vi "Get stack field.vi"(7 "Is Module?":bool, 8 "error in (no error)":errorcluster, 10 "Field":string, 11 "Stack in":refnum<class "Stack.lvclass">) -> (0 "error out":errorcluster, 1 "Value out":string, 3 "Stack out":refnum<class "Stack.lvclass">)   [LabVIEW 2021, in "Stack.lvclass"]
uses:
  Stack.lvclass
  Stack.lvclass/Stack.ctl
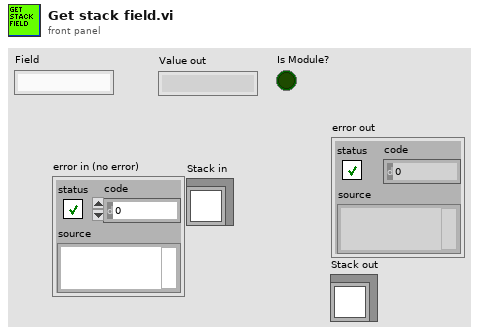
[diagram p1: front panel]
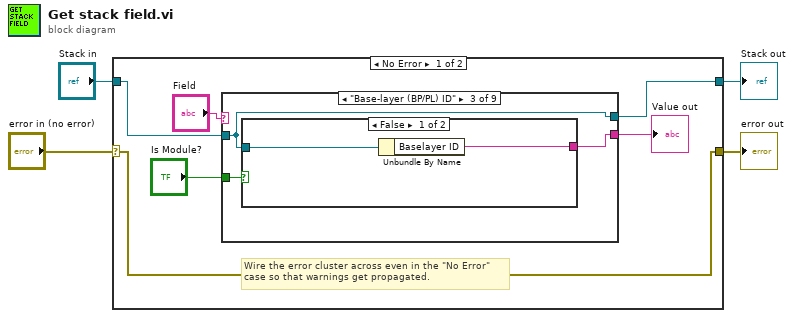
[diagram p0: block diagram]
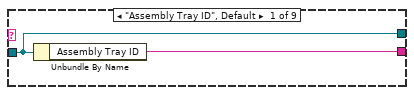
[diagram p2: hidden frame]
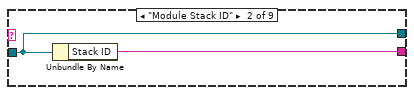
[diagram p3: hidden frame]
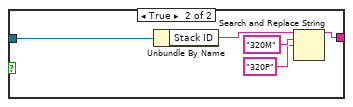
[diagram p4: hidden frame]
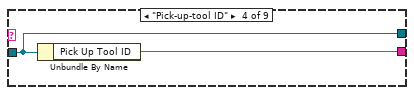
[diagram p5: hidden frame]
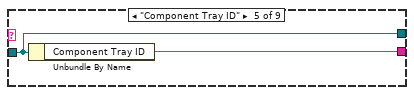
[diagram p6: hidden frame]
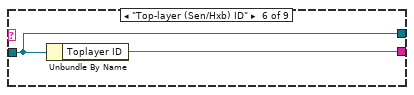
[diagram p7: hidden frame]
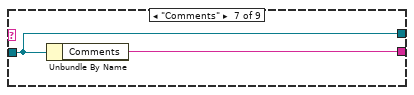
[diagram p8: hidden frame]
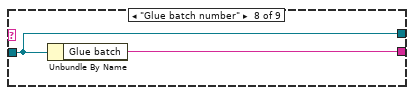
[diagram p9: hidden frame]
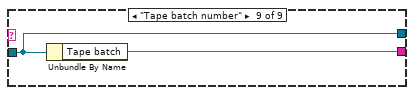
[diagram p10: hidden frame]
diagram:
  n1 = case shown="No Error" "error in (no error)" {
    selector: "error in (no error)" -> [w10 w38]
    tunnel: [w10 w38] -> w3
    tunnel: [w8 w37] -> w1
    tunnel: "Stack in" -> [w9 w37]
    frame No Error {
      # "Wire the error cluster across even in the \"No Error\"\ncase so that warnings get propagated."
      n2 = case shown="\"Base-layer (BP/PL) ID\"" "Field" {
        tunnel: w9 -> [w12 w13 w16 w26 w28 w30 w32 w34 w36]
        tunnel: [w12 w13 w16 w26 w28 w30 w32 w34 w36] -> w8
        tunnel: [w11 w14 w15 w25 w27 w29 w31 w33 w35] -> w6
        tunnel: "Is Module?" -> [_ _ w17 _ _ _ _ _ _]
        frame "Assembly Tray ID", Default {
          n3 = Unbundle By Name(w12) -> ("Assembly Tray ID"=w11:string)
        }
        frame "Module Stack ID" {
          n4 = Unbundle By Name(w13) -> ("Stack ID"=w14:string)
        }
        frame "Base-layer (BP/PL) ID" {
          n5 = case shown="False" w17 {
            tunnel: w16 -> [w19 w24]
            tunnel: [w18 w20] -> w15
            frame False {
              n6 = Unbundle By Name(w19) -> ("Baselayer ID"=w18:string)
            }
            frame True {
              n7 = Unbundle By Name(w24) -> ("Stack ID"=w21:string)
              n8 = Search and Replace String(input string=w21, search string="320M", replace string="320P" ("replace string (\"\")")) -> (result string=w20:string)  [unwired: 5 in, 3 out]
            }
          }
        }
        frame "Pick-up-tool ID" {
          n9 = Unbundle By Name(w26) -> ("Pick Up Tool ID"=w25:string)
        }
        frame "Component Tray ID" {
          n10 = Unbundle By Name(w28) -> ("Component Tray ID"=w27:string)
        }
        frame "Top-layer (Sen/Hxb) ID" {
          n11 = Unbundle By Name(w30) -> ("Toplayer ID"=w29:string)
        }
        frame "Comments" {
          n12 = Unbundle By Name(w32) -> ("Comments"=w31:string)
        }
        frame "Glue batch number" {
          n13 = Unbundle By Name(w34) -> ("Glue batch"=w33:string)
        }
        frame "Tape batch number" {
          n14 = Unbundle By Name(w36) -> ("Tape batch"=w35:string)
        }
      }
      "Value out" <- w6
    }
    frame Error {
    }
  }
  "error out" <- w3
  "Stack out" <- w1
